vi "LTVDiffDriveCtrl_AtReference.vi"(11 "LTV_DIFF_DRIVE_CTRL":T1) -> (3 "At Reference":bool)   [LabVIEW 2019, in "Trajectory_Library.lvlib"]
doc: "Returns true if the pose error is within tolerance of the reference.\n\nInputs:\n - LTV Diff Drive Ctrl -- Controller data cluster\n\nOutputs:\n - At Reference -- True if the pose error is within tolerance of the reference."
uses:
  Trajectory_Library.lvlib
  TypeDef/LTV_DIFF_DRIVE_CTRL.ctl
  TypeDef/FUNCTION_GENERATOR_MATRIX.ctl
  <vilib>/Analysis/Matrix/Datatypes/RealMatrix.ctl
  <vilib>/Analysis/Matrix/NI_Matrix.lvlib
panel:
  # "< 5, 1 >"
  # "< 5, 1 >"
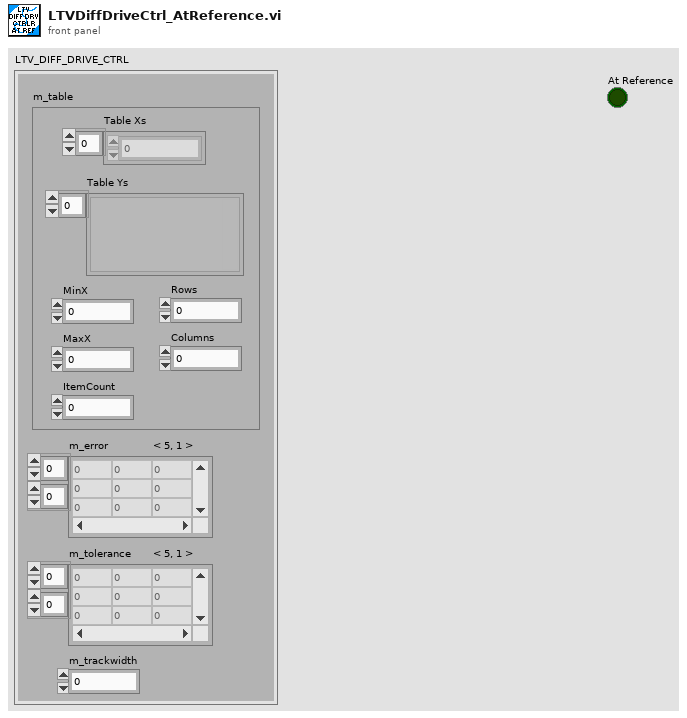
[diagram p1: front panel]
types:
  T1 = typedef "Trajectory_Library.lvlib/LTV_DIFF_DRIVE_CTRL.ctl" = cluster{"m_table":T2, "m_error":T3, "m_tolerance":T3, "m_trackwidth":dbl}
  T2 = typedef "Trajectory_Library.lvlib/FUNCTION_GENERATOR_MATRIX.ctl" = cluster{"Table Xs":dbl[], "Table Ys":variant[], "MinX":dbl, "MaxX":dbl, "ItemCount":i32, "Rows":i32, "Columns":i32}
  T3 = typedef "NI_Matrix.lvlib/RealMatrix.ctl" = dbl[][]
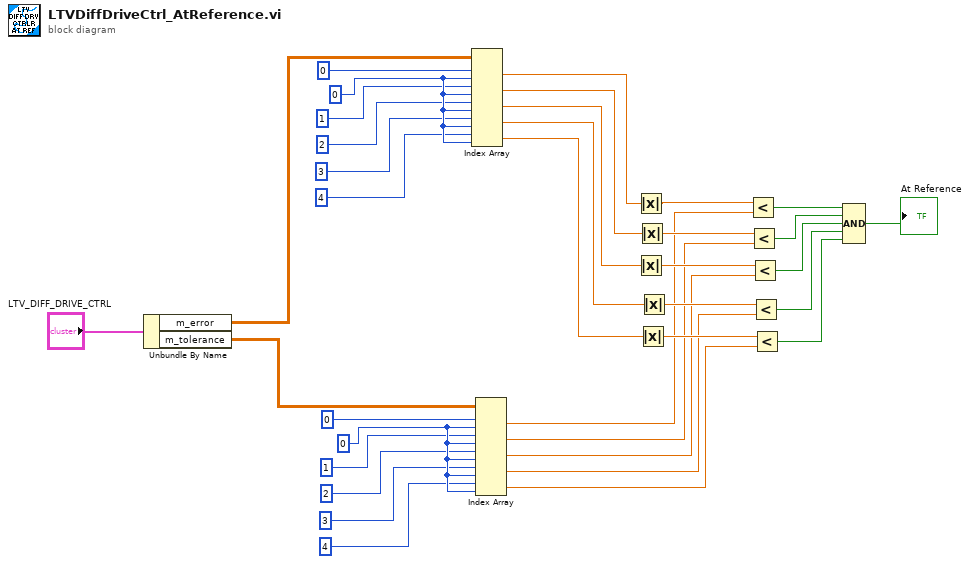
[diagram p0: block diagram]
diagram:
  w11 = 0 ("index (col)")
  w17 = 0 ("index (col)")
  n1 = Unbundle By Name("LTV_DIFF_DRIVE_CTRL") -> ("m_error"=w23:T3, "m_tolerance"=w6:T3)
  n2 = Index Array(array=w23, index (row) #1=0 ("index (row)"), index (col) #1=w17, index (row) #2=1 ("index (row)"), index (col) #2=w17, index (row) #3=2 ("index (row)"), index (col) #3=w17, index (row) #4=3 ("index (row)"), index (col) #4=w17, index (row) #5=4 ("index (row)"), index (col) #5=w17) -> (element #1=w22:dbl, element #2=w21:dbl, element #3=w20:dbl, element #4=w19:dbl, element #5=w18:dbl)
  n3 = Index Array(array=w6, index (row) #1=0 ("index (row)"), index (col) #1=w11, index (row) #2=1 ("index (row)"), index (col) #2=w11, index (row) #3=2 ("index (row)"), index (col) #3=w11, index (row) #4=3 ("index (row)"), index (col) #4=w11, index (row) #5=4 ("index (row)"), index (col) #5=w11) -> (element #1=w5:dbl, element #2=w4:dbl, element #3=w3:dbl, element #4=w2:dbl, element #5=w1:dbl)
  n4 = Absolute Value(x=w22) -> (abs(x)=w35:dbl)
  n5 = Absolute Value ("Absolute Value.vi")(x=w20) -> (abs(x)=w33:dbl)
  n6 = Absolute Value ("Absolute Value.vi")(x=w21) -> (abs(x)=w34:dbl)
  n7 = Absolute Value ("Absolute Value.vi")(x=w18) -> (abs(x)=w27:dbl)
  n8 = Absolute Value ("Absolute Value.vi")(x=w19) -> (abs(x)=w28:dbl)
  n9 = Less?(x=w35, y=w5) -> (x < y?=w32:bool)
  n10 = Less?(x=w34, y=w4) -> (x < y?=w31:bool)
  n11 = Less?(x=w33, y=w3) -> (x < y?=w30:bool)
  n12 = Less?(x=w28, y=w2) -> (x < y?=w26:bool)
  n13 = Less?(x=w27, y=w1) -> (x < y?=w25:bool)
  n14 = Compound Arithmetic op=AND(w32, w31, w30, w26, w25) -> (→"At Reference":bool)
